vi "buildStringTable.vi"(1 "column headers":string[](array[string]), 2 "row headers":string[](array[string]), 3 "text data":string[][](array[string])) -> (0 "output table":string[][](array[string]))   [LabVIEW 2017, in "LabVIEW NPOI.lvlib" / "Document.lvclass"]
uses:
  Document.lvclass
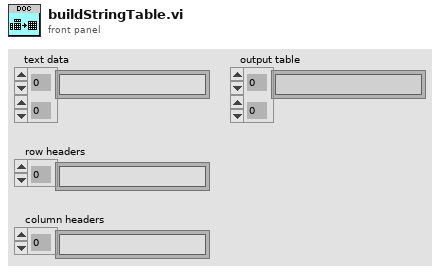
[diagram p1: front panel]
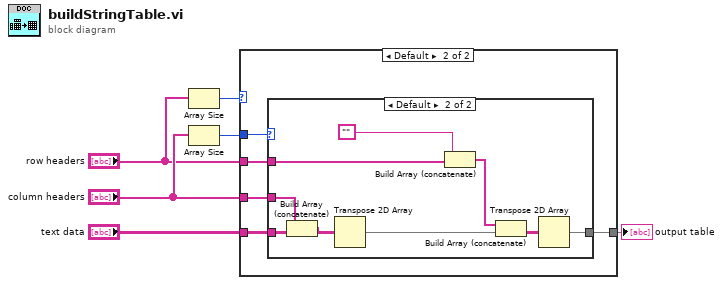
[diagram p0: block diagram]
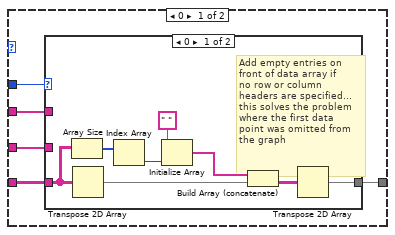
[diagram p2: hidden frame]
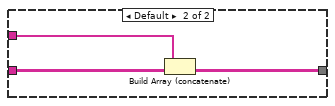
[diagram p3: hidden frame]
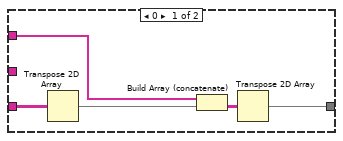
[diagram p4: hidden frame]
diagram:
  n1 = Array Size(array="row headers") -> (size(s)=w1:i32)
  n2 = Array Size(array="column headers") -> (size(s)=w2:i32)
  n3 = case shown="Default" w1 {
    tunnel: "text data" -> [w11 w26]
    tunnel: "column headers" -> [w10 w25]
    tunnel: "row headers" -> [w9 w27]
    tunnel: [w8 w23] -> w3
    tunnel: w2 -> [w7 w24]
    frame 0 {
      n4 = case shown="0" w7 {
        tunnel: w10 -> [_ w22]
        tunnel: w11 -> [w16 w21]
        tunnel: [w17 w20] -> w8
        tunnel: w9 -> [_ _]
        frame 0 {
          # "Add empty entries on\nfront of data array if\nno row or column \nheaders are specified...\nthis solves the problem\nwhere the first data \npoint was omitted from\nthe graph"
          n5 = Array Size(array=w16) -> (size(s)=w15:i32[])
          n6 = Transpose 2D Array(2D array=w16) -> (transposed array=w18:string[][])
          n7 = Index Array(array=w15) -> (element=w14:i32)  [unwired: 1 in]
          n8 = Initialize Array(" ", w14) -> (w13:string[])
          n9 = Build Array (concatenate)(w13, w18) -> (w19:string[][])
          n10 = Transpose 2D Array(2D array=w19) -> (transposed array=w17:string[][])
        }
        frame Default {
          n11 = Build Array (concatenate)(w22, w21) -> (w20:string[][])
        }
      }
    }
    frame Default {
      n12 = case shown="Default" w24 {
        tunnel: [w29 w39] -> w23
        tunnel: w25 -> [_ w36]
        tunnel: w26 -> [w31 w35]
        tunnel: w27 -> [w32 w33]
        frame 0 {
          n13 = Transpose 2D Array(2D array=w31) -> (transposed array=w30:string[][])
          n14 = Build Array (concatenate)(w32, w30) -> (w28:string[][])
          n15 = Transpose 2D Array(2D array=w28) -> (transposed array=w29:string[][])
        }
        frame Default {
          n16 = Build Array (concatenate)(w36, w35) -> (w34:string[][])
          n17 = Transpose 2D Array(2D array=w34) -> (transposed array=w38:string[][])
          n18 = Build Array (concatenate)("", w33) -> (w37:string[])
          n19 = Build Array (concatenate)(w37, w38) -> (w40:string[][])
          n20 = Transpose 2D Array(2D array=w40) -> (transposed array=w39:string[][])
        }
      }
    }
  }
  "output table" <- w3
